vi "Native_AddCaseFrame_v2.vi"() -> ()   [LabVIEW 2024]
panel:
  out "error out":errorcluster caption="错误输出"
  out "frame_id":u32
  in  "frame_id type":u32
  in  "after":bool
  in  "reference_frame_index":u32
  in  "case_id":u32
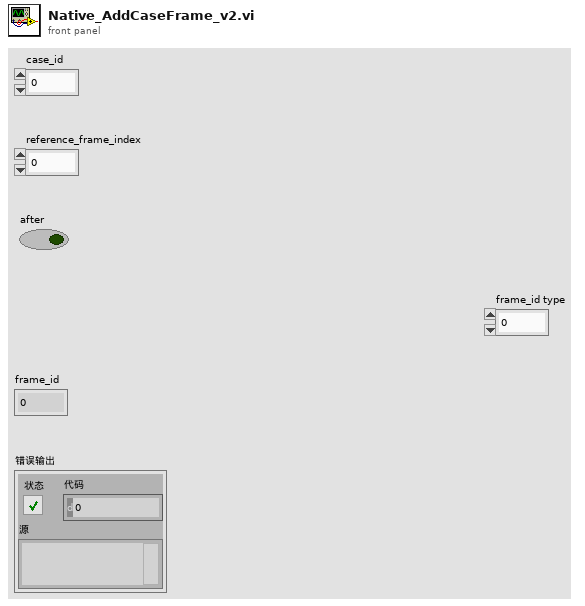
[diagram p1: front panel]
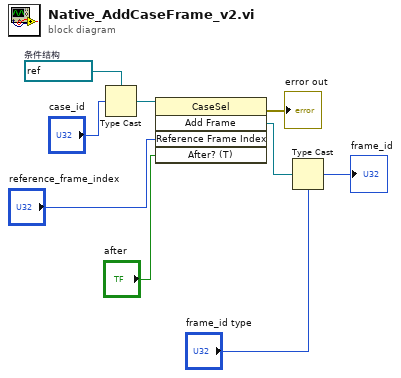
[diagram p0: block diagram]
diagram:
  w8 = refnum<vi> refnum  # 条件结构
  n1 = Type Cast ("强制类型转换")(type=w8, x="case_id") -> (*(type *) &x=w7:refnum<vi>)
  n2 = invoke class="CaseSel" method="Add Frame"(reference=w7, "Reference Frame Index"="reference_frame_index", "After? (T)"="after") -> (error out=→"error out":errorcluster, "Add Frame"=w4:refnum<vi>)  [unwired: 2 in, 3 out]
  n3 = Type Cast ("强制类型转换")(type="frame_id type", x=w4) -> (*(type *) &x=→"frame_id":u32)
